vi "Actividad Termometros-Mateo Cuaspud.vi"() -> ()   [LabVIEW 2026]
panel:
  out "CALIENTE":bool
  out "FRIO":bool
  in  "stop":bool
  out "°K":dbl(slide) scale=0.0..500.0
  out "°F":dbl(slide) scale=0.0..500.0
  out "°C":dbl(slide) scale=0.0..500.0
  in  "Slide":dbl(slide) scale=0.0..500.0
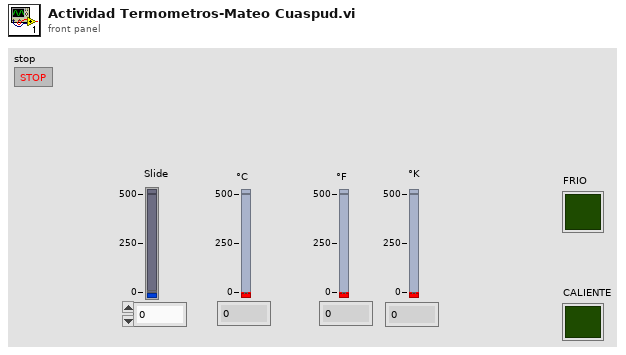
[diagram p1: front panel]
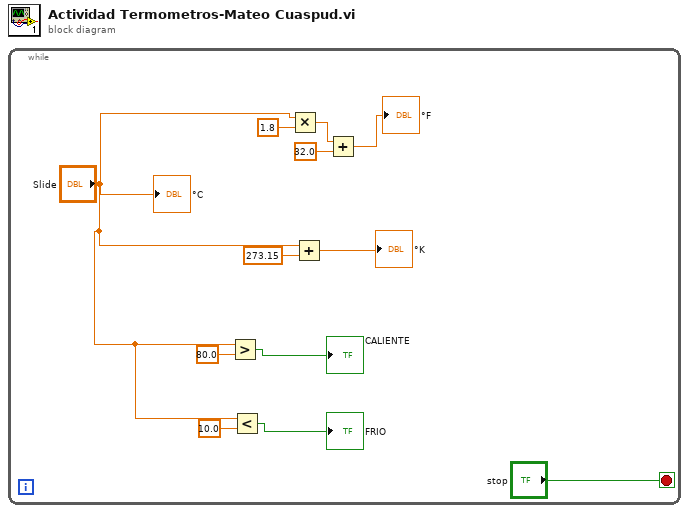
[diagram p0: block diagram]
diagram:
  n1 = while {
    stop <- "stop" stop-if-true
    n2 = Greater?(x="Slide", y=80.0) -> (0:→"CALIENTE":bool)
    n3 = Less?(x="Slide", y=10.0) -> (x < y?=→"FRIO":bool)
    n4 = Multiply(x="Slide", y=1.8) -> (x*y=w10:dbl)
    n5 = Add(x="Slide", y=273.15) -> (x+y=→"°K":dbl)
    n6 = Add(x=w10, y=32.0) -> (x+y=→"°F":dbl)
    "°C" <- "Slide"
  }
